vi "simulate camera image.vi"(8 "error in (no error)":errorcluster, 11 "FakeCamera in":refnum<class "Point Grey Camera.lvclass">) -> (0 "error out":errorcluster, 2 "Acquisition OK?":bool, 3 "FakeCamera out":refnum<class "Point Grey Camera.lvclass">, 5 "acq time (ms)":u32)   [LabVIEW 2020, in "Point Grey Camera.lvclass"]
uses:
  Point Grey Camera.lvclass
  Point Grey Camera.lvclass/Point Grey Camera.ctl
  NI_Vision_Development_Module.lvlib
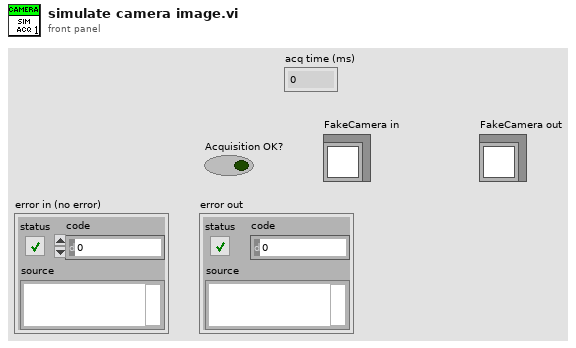
[diagram p1: front panel]
types:
  T1 = typedef "IMAQ Image.ctl" = refnum<image>
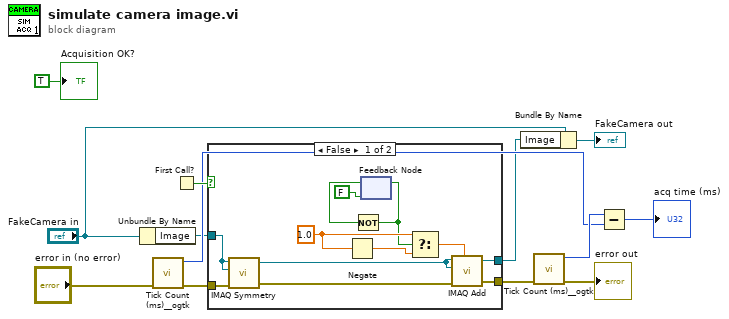
[diagram p0: block diagram]
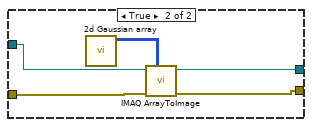
[diagram p2: hidden frame]
diagram:
  n1 = Unbundle By Name("FakeCamera in") -> ("Image"=w4:T1)
  n2 = call "Tick Count (ms)__ogtk.vi"("error in (no error)"="error in (no error)") -> ("error out"=w6:errorcluster, "millisecond timer value"=w8:u32)  [unwired: 9 in]
  n3 = First Call?() -> (First Call?: T/F=w13:bool)
  n4 = case shown="False" w13 {
    tunnel: w6 -> [w24 w30]
    tunnel: [w15 w29] -> w11
    tunnel: [w16 w28] -> w3
    tunnel: w4 -> [w25 w27]
    frame False {
      w20 = 1.0 ("Constant")
      n5 = call "IMAQ Symmetry"("error in (no error)"=w24, "Image Dst"=w25, "Image Src"=w25) -> ("error out"=w14:errorcluster, "Image Dst Out"=w23:T1)  [unwired: 2 in]
      n6 = Negate(x=w20) -> (-x=w19:dbl)
      n7 = feedback #1(FALSE) -> (w22:bool)
      n8 = Not(x=w22) -> (.not. x?=w18:bool)
      n9 = feedback-in #1(w18) -> ()
      n10 = Select(t=w20, s=w18, f=w19) -> (s? t:f=w17:dbl)
      n11 = call "IMAQ Add"("Image Src A"=w23, "Constant"=w17, "Image Dst"=w23, "error in (no error)"=w14) -> ("Image Dst Out"=w16:T1, "error out"=w15:errorcluster)  [unwired: 3 in]
    }
    frame True {
      n12 = call "2d Gaussian array.vi"() -> ("Intensity Graph"=w26:u16[][])  [unwired: 11 in]
      n13 = call "IMAQ ArrayToImage"("Image Pixels (U16)"=w26, "error in (no error)"=w30, "Image"=w27) -> ("error out"=w29:errorcluster, "Image Out"=w28:T1)  [unwired: 7 in]
    }
  }
  n14 = Bundle By Name(cluster="FakeCamera in", "Image"=w3) -> (→"FakeCamera out":refnum<class "Point Grey Camera.lvclass">)
  n15 = call "Tick Count (ms)__ogtk.vi"("error in (no error)"=w11) -> ("error out"=→"error out":errorcluster, "millisecond timer value"=w9:u32)  [unwired: 9 in]
  n16 = Subtract(x=w9, y=w8) -> (x-y=→"acq time (ms)":u32)
  "Acquisition OK?" <- TRUE ("Acquisition OK?")
